vi "MatrixMultiblock.vi"(7 "Induction Matrix Build Properties":T2, 11 "Port States In":T1) -> (3 "Port States Out":T1)   [LabVIEW 2026]
uses:
  Induction Matrix Build Properties.ctl
  Port Defs/Matrix Port States.ctl
panel:
  out "Energy (FE)":ext(slide) scale=-1.0..25600000000.0 scale format="%#_12f"
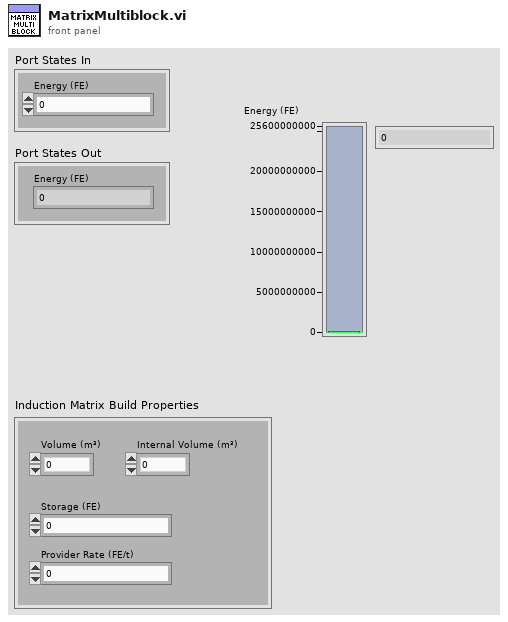
[diagram p1: front panel]
types:
  T1 = typedef "Matrix Port States.ctl" = cluster{"Energy (FE)":ext}
  T2 = typedef "Induction Matrix Build Properties.ctl" = cluster{"Internal Volume (m³)":i32, "Volume (m³)":i32, "Storage (FE)":ext, "Provider Rate (FE/t)":ext}
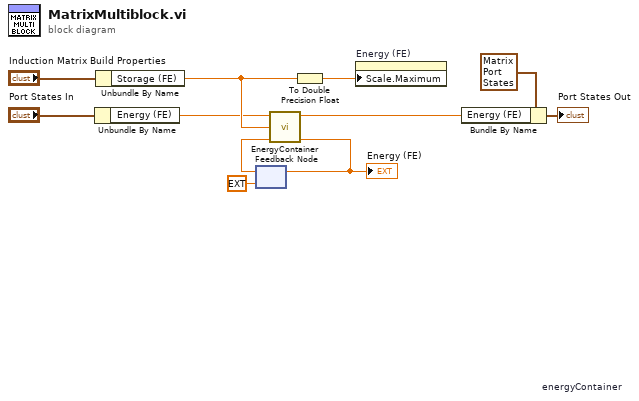
[diagram p0: block diagram]
diagram:
  n1 = Unbundle By Name("Port States In") -> ("Energy (FE)"=w4:ext)
  n2 = Unbundle By Name("Induction Matrix Build Properties") -> ("Storage (FE)"=w6:ext)
  n3 = feedback #1 "energyContainer"(ext 0.0 ("Fill (FE)")) -> (w11:ext)
  n4 = call "EnergyContainer.vi"("Capacity (FE)"=w6, "Last Fill (FE)"=w11, "Transfer (FE)"=w4) -> ("Fill (FE)"=w9:ext, "Overflow (FE)"=w1:ext)  [unwired: 2 in, 2 out]
  "Energy (FE)" <- w9
  n5 = feedback-in #1(w9) -> ()
  n6 = To Double Precision Float(number=w6) -> (double precision float=w8:dbl)
  n7 = property on="Energy (FE)" class="Slide (strict)"("Scale.Maximum"=w8) -> ()  [unwired: 2 in, 2 out]
  n8 = Bundle By Name(cluster=T1 {"Energy (FE)"=0.0} ("Induction Matrix Port States"), "Energy (FE)"=w1) -> (→"Port States Out":T1)
